vi "shear_and_recovery__87515e5cab.vi"(7 "real strain":dbl[](array[numeric]), 8 "recovery strain":dbl[](array[numeric]), 9 "Gap":dbl, 10 "voltage to displacement contant":dbl, 11 "initial position in voltage":dbl) -> (2 "real strain (-)":dbl[](array[numeric]), 3 "recovery strain (-)":dbl[](array[numeric]))   [LabVIEW 2023]
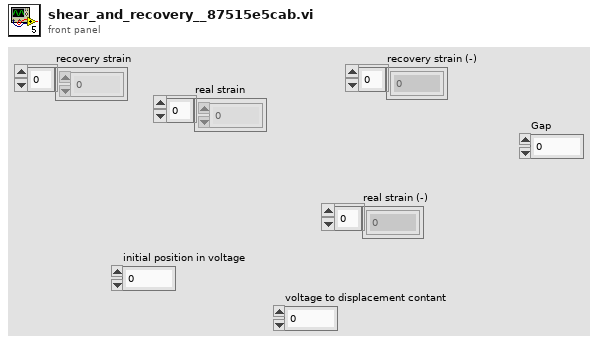
[diagram p1: front panel]
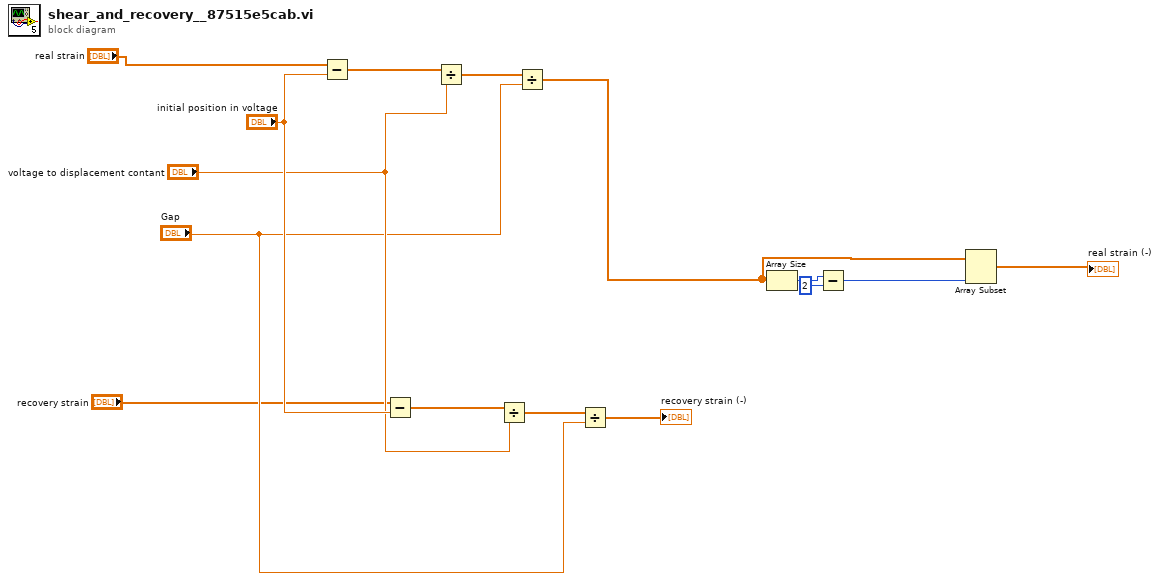
[diagram p0: block diagram]
diagram:
  n1 = Subtract(x="real strain", y="initial position in voltage") -> (x-y=w14:dbl[])
  n2 = Subtract(x="recovery strain", y="initial position in voltage") -> (x-y=w11:dbl[])
  n3 = Divide(x=w14, y="voltage to displacement contant") -> (x/y=w15:dbl[])
  n4 = Divide(x=w11, y="voltage to displacement contant") -> (x/y=w12:dbl[])
  n5 = Divide(x=w15, y="Gap") -> (x/y=w3:dbl[])
  n6 = Divide(x=w12, y="Gap") -> (x/y=→"recovery strain (-)":dbl[])
  n7 = Array Size(array=w3) -> (size(s)=w6:i32)
  n8 = Subtract(x=w6, y=2) -> (x-y=w4:i32)
  n9 = Array Subset(array=w3, length=w4) -> (→"real strain (-)":dbl[])  [unwired: 1 in]
